vi "RemoteVI Thread Windows.vi"(0 "hWnd":u64, 11 "error in":errorcluster) -> (4 "active":u64, 6 "focus":u64, 8 "capture":u64, 15 "error out":errorcluster)   [LabVIEW 2020, in "RemoteVI.lvlib"]
doc: "Which windows of the GUI thread that owns hWnd (LabVIEW's UI thread) are active, have the keyboard focus and hold the mouse capture right now: user32 GetWindowThreadProcessId.vi, then user32 GetGUIThreadInfo.vi with the 64-bit GUITHREADINFO (cbSize 72, each HWND two U32, low first: hwndActive [2,3], hwndFocus [4,5], hwndCapture [6,7]); when that call fails it is repeated with the 32-bit layout (cbSize 48, one U32 each: [2], [3], [4]). Both run in any thread, so this answers while a dialog or a popup holds the UI thread in its modal loop. The focus window can be a CHILD window - the file name box of a native file dialog. A window that does not exist gives 0. An incoming error skips the work."
uses:
  RemoteVI.lvlib
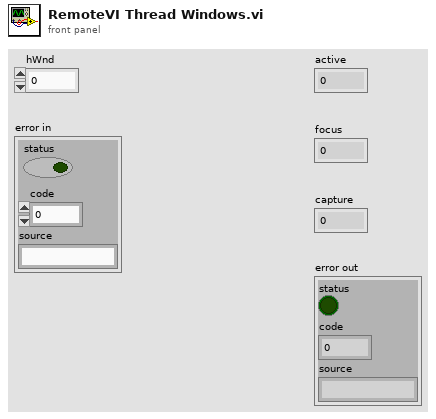
[diagram p1: front panel]
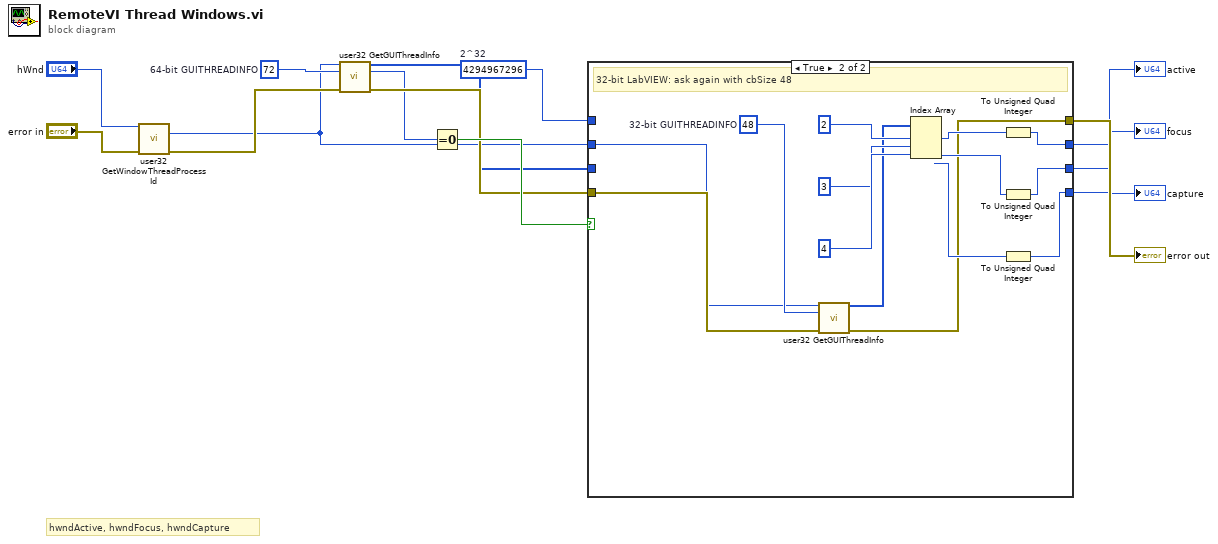
[diagram p0: block diagram]
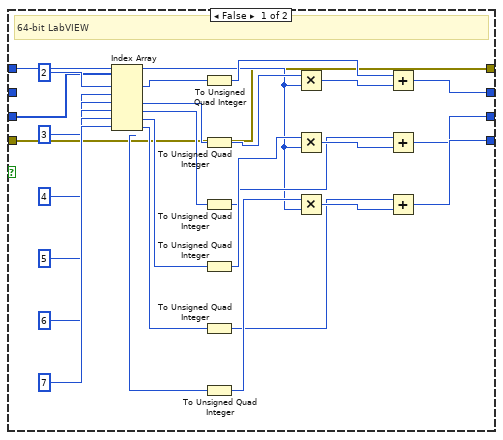
[diagram p2: hidden frame]
diagram:
  w10 = u64 4294967296  # 2^32
  w5 = u32 72  # 64-bit GUITHREADINFO
  # "hwndActive, hwndFocus, hwndCapture"
  n1 = call "user32 GetWindowThreadProcessId.vi"("hWnd"="hWnd", "error in"="error in") -> ("thread ID"=w3:u32, "error out"=w4:errorcluster)  [unwired: 11 in, 1 out]
  n2 = call "user32 GetGUIThreadInfo.vi"("thread ID"=w3, "cbSize"=w5, "error in"=w4) -> ("info"=w6:u32[], "return value"=w7:i32, "error out"=w8:errorcluster)  [unwired: 10 in]
  n3 = Equal To 0?(x=w7) -> (x = 0?=w9:bool)
  n4 = case shown="True" w9 {
    tunnel: w10 -> [w17 _]
    tunnel: w3 -> [_ w42]
    tunnel: w6 -> [w15 _]
    tunnel: w8 -> [w16 w43]
    tunnel: [w16 w46] -> w14
    tunnel: [w39 w53] -> w11
    tunnel: [w40 w54] -> w12
    tunnel: [w41 w55] -> w13
    frame False {
      # "64-bit LabVIEW"
      n5 = Index Array(array=w15, index #1=2, index #2=3, index #3=4, index #4=5, index #5=6, index #6=7) -> (element #1=w24:u32, element #2=w25:u32, element #3=w26:u32, element #4=w27:u32, element #5=w28:u32, element #6=w29:u32)
      n6 = To Unsigned Quad Integer(1:w24) -> (0:w30:u64)
      n7 = To Unsigned Quad Integer(1:w25) -> (0:w31:u64)
      n8 = To Unsigned Quad Integer(1:w26) -> (0:w32:u64)
      n9 = To Unsigned Quad Integer(1:w27) -> (0:w33:u64)
      n10 = To Unsigned Quad Integer(1:w28) -> (0:w34:u64)
      n11 = To Unsigned Quad Integer(1:w29) -> (0:w35:u64)
      n12 = Multiply(x=w31, y=w17) -> (x*y=w36:u64)
      n13 = Multiply(x=w33, y=w17) -> (x*y=w37:u64)
      n14 = Multiply(x=w35, y=w17) -> (x*y=w38:u64)
      n15 = Add(x=w30, y=w36) -> (x+y=w39:u64)
      n16 = Add(x=w32, y=w37) -> (x+y=w40:u64)
      n17 = Add(x=w34, y=w38) -> (x+y=w41:u64)
    }
    frame True {
      w44 = u32 48  # 32-bit GUITHREADINFO
      # "32-bit LabVIEW: ask again with cbSize 48"
      n18 = call "user32 GetGUIThreadInfo.vi"("thread ID"=w42, "cbSize"=w44, "error in"=w43) -> ("info"=w45:u32[], "error out"=w46:errorcluster)  [unwired: 10 in, 1 out]
      n19 = Index Array(array=w45, index #1=2, index #2=3, index #3=4) -> (element #1=w50:u32, element #2=w51:u32, element #3=w52:u32)
      n20 = To Unsigned Quad Integer(1:w50) -> (0:w53:u64)
      n21 = To Unsigned Quad Integer(1:w51) -> (0:w54:u64)
      n22 = To Unsigned Quad Integer(1:w52) -> (0:w55:u64)
    }
  }
  "active" <- w11
  "focus" <- w12
  "capture" <- w13
  "error out" <- w14
